vi "VIH Platform - LabVIEW - Palette - Get Item Image.vi"(8 "error in":errorcluster, 11 "Palette Item Name":string) -> (0 "error out":errorcluster, 2 "Palette Item Icon":T1, 3 "dup Palette Item Name":string)   [LabVIEW 2014]
doc: "::: VI Helpeks :::\nCopyright (c) 2000-2026 Konstantin Shifershteyn. All rights reserved."
uses:
  <vilib>/picture/picture.llb/imagedata.ctl
panel:
  # "VI Helpeks\nCopyright (c) 2012-2026 Konstantin Shifershteyn"
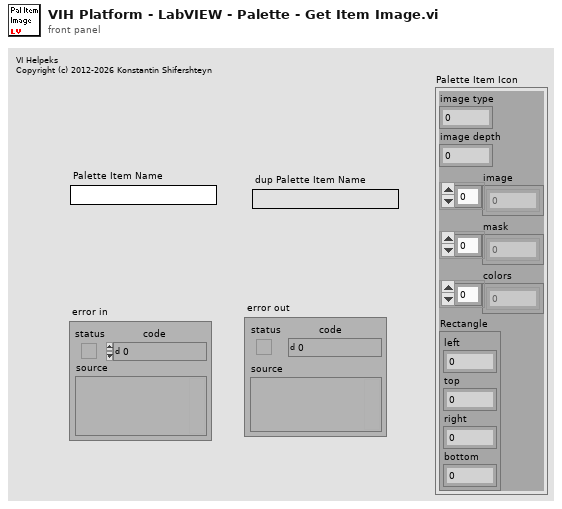
[diagram p1: front panel]
types:
  T1 = typedef "imagedata.ctl" = cluster{"image type":i32, "image depth":i32, "image":u8[], "mask":u8[], "colors":u32[], "Rectangle":cluster{"left":i16, "top":i16, "right":i16, "bottom":i16}}
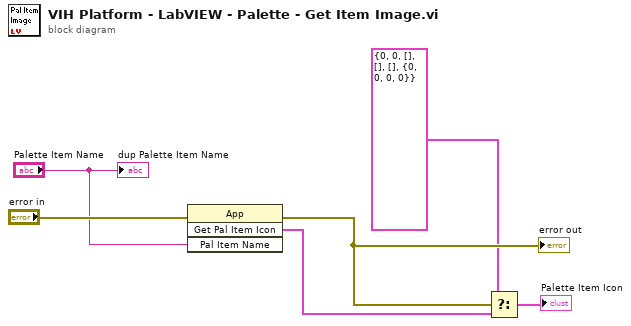
[diagram p0: block diagram]
diagram:
  n1 = invoke class="App" method="Get Pal Item Icon"(error in="error in", "Pal Item Name"="Palette Item Name") -> (error out=w5:errorcluster, "Get Pal Item Icon"=w2:T1)  [unwired: 2 in, 2 out]
  "error out" <- w5
  n2 = Select(t=T1 {"image type"=0, "image depth"=0, "image"=[], "mask"=[], "colors"=[], "Rectangle"={"left"=0, "top"=0, "right"=0, "bottom"=0}} ("Palettes:Get Palette Item Icon"), s=w5, f=w2) -> (s? t:f=→"Palette Item Icon":T1)
  "dup Palette Item Name" <- "Palette Item Name"
